vi "OwnInterface20261013_AddParent.vi"() -> ()   [LabVIEW 2024]
panel:
  out "error out":errorcluster caption="错误输出"
  in  "Save Class Path":path
  in  "Interface Path":path
  in  "Class Path":path
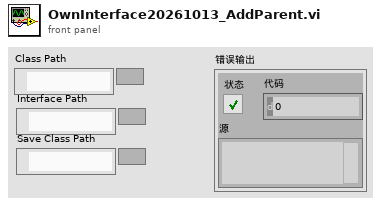
[diagram p1: front panel]
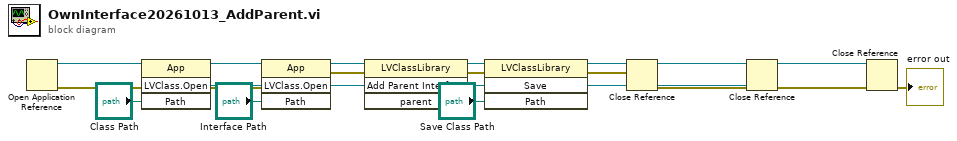
[diagram p0: block diagram]
diagram:
  n1 = Open Application Reference() -> (0:w12:errorcluster, 3:w14:refnum<vi>)  [unwired: 4 in]
  n2 = invoke class="App" method="LVClass.Open"(reference=w14, error in=w12, "Path"="Class Path") -> ("LVClass.Open"=w10:refnum<vi>)  [unwired: 1 in, 3 out]
  n3 = invoke class="App" method="LVClass.Open"(reference=w14, error in=w12, "Path"="Interface Path") -> (error out=w8:errorcluster, "LVClass.Open"=w9:refnum<vi>)  [unwired: 1 in, 2 out]
  n4 = invoke class="LVClassLibrary" method="Add Parent Interface"(reference=w10, error in=w8, "parent"=w9) -> (reference out=w7:refnum<vi>, error out=w5:errorcluster)  [unwired: 1 in, 2 out]
  n5 = invoke class="LVClassLibrary" method="Save"(reference=w7, error in=w5, "Path"="Save Class Path") -> (error out=w4:errorcluster)  [unwired: 1 in, 3 out]
  n6 = Close Reference(reference=w9, error in (no error)=w4) -> (error out=w3:errorcluster)
  n7 = Close Reference(reference=w10, error in (no error)=w3) -> (error out=w2:errorcluster)
  n8 = Close Reference(reference=w14, error in (no error)=w2) -> (error out=→"error out":errorcluster)
